vi "Update Table Buffer Pressure.vi"(7 "BUFFER Ref":refnum<vi>, 8 "error in (no error)":errorcluster, 11 "Table Buffer Pressure Ref":refnum<vi>) -> (0 "error out":errorcluster)   [LabVIEW 2025, in "I2C Bus Monitor UI.lvlib"]
uses:
  I2C Bus Monitor UI.lvlib
  Table Buffer - Check.vi
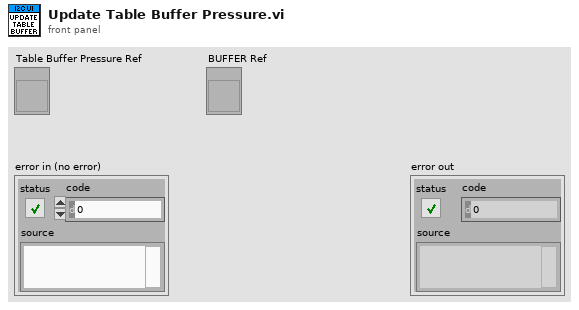
[diagram p1: front panel]
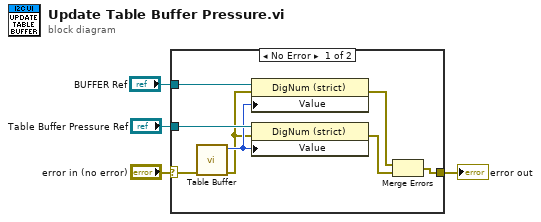
[diagram p0: block diagram]
diagram:
  n1 = case shown="No Error" "error in (no error)" {
    selector: "error in (no error)" -> [w12 w13]
    tunnel: "Table Buffer Pressure Ref" -> [w10 _]
    tunnel: "BUFFER Ref" -> [w9 _]
    tunnel: [w7 w13] -> w1
    frame No Error {
      n2 = call-poly "Table Buffer.vi"("error in (no error)"=w12) -> ("error out"=w5:errorcluster, "# Elements in Buffer"=w8:i32)  [unwired: 8 in, 1 out]
      n3 = property class="DigNum (strict)"(reference=w9, error in=w5, "Value"=w8) -> (error out=w6:errorcluster)  [unwired: 1 out]
      n4 = property class="DigNum (strict)"(reference=w10, error in=w5, "Value"=w8) -> (error out=w11:errorcluster)  [unwired: 1 out]
      n5 = Merge Errors(w6, w11) -> (w7:errorcluster)
    }
    frame Error {
    }
  }
  "error out" <- w1
